vi "CilindarTest.vi"() -> ()   [LabVIEW 2014]
panel:
  out "Boolean 7":bool
  out "Boolean 6":bool
  out "Boolean 5":bool
  out "Boolean 4":bool
  out "Boolean 3":bool
  out "Boolean 2":bool
  out "Boolean":bool
  in  "stop":bool
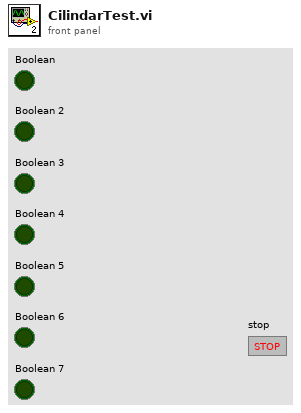
[diagram p1: front panel]
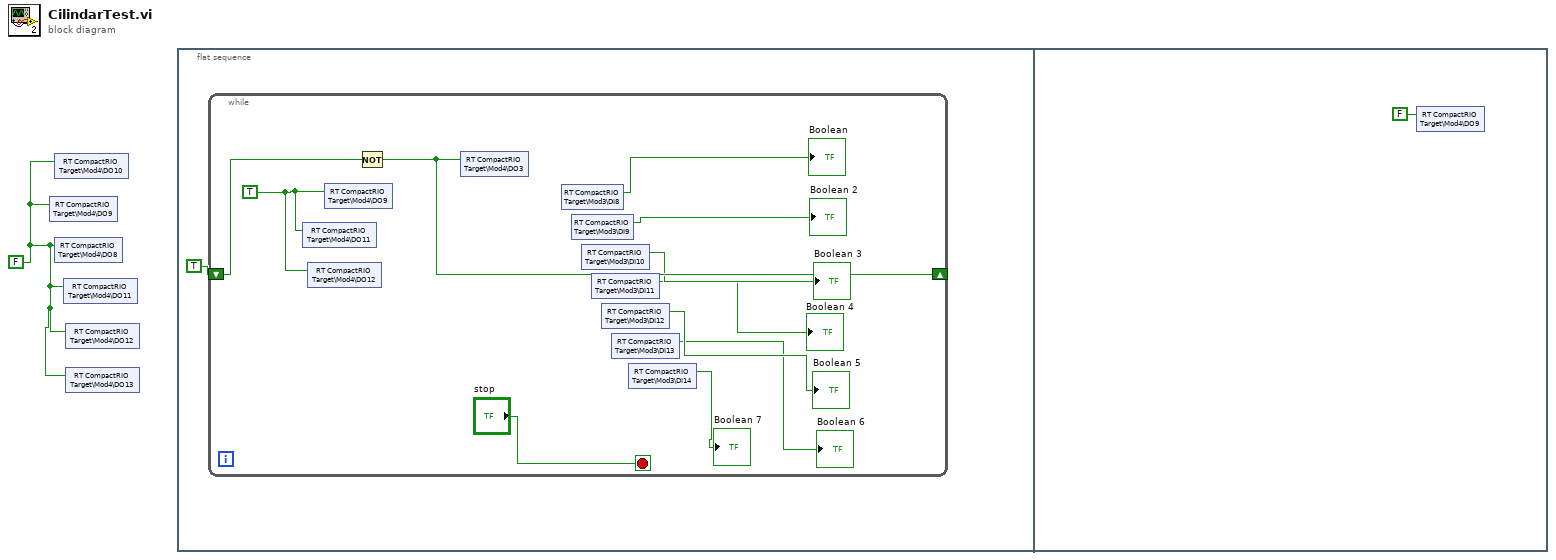
[diagram p0: block diagram]
diagram:
  w1 = FALSE
  n1 = shared-variable "RT CompactRIO Target\\Mod4\\DO9"(w1) -> ()  [unwired: 1 in, 1 out]
  n2 = shared-variable "RT CompactRIO Target\\Mod4\\DO10"(w1) -> ()  [unwired: 1 in, 1 out]
  n3 = shared-variable "RT CompactRIO Target\\Mod4\\DO8"(w1) -> ()  [unwired: 1 in, 1 out]
  n4 = shared-variable "RT CompactRIO Target\\Mod4\\DO11"(w1) -> ()  [unwired: 1 in, 1 out]
  n5 = shared-variable "RT CompactRIO Target\\Mod4\\DO12"(w1) -> ()  [unwired: 1 in, 1 out]
  n6 = shared-variable "RT CompactRIO Target\\Mod4\\DO13"(w1) -> ()  [unwired: 1 in, 1 out]
  n7 = flat-sequence {
    frame #0 {
      n8 = while {
        shift-right: [w12] -> _
        shift-left: TRUE ("DO8") -> [w13]
        stop <- "stop" stop-if-true
        w11 = TRUE ("DO8")
        n9 = shared-variable "RT CompactRIO Target\\Mod4\\DO11"(w11) -> ()  [unwired: 1 in, 1 out]
        n10 = shared-variable "RT CompactRIO Target\\Mod4\\DO12"(w11) -> ()  [unwired: 1 in, 1 out]
        n11 = shared-variable "RT CompactRIO Target\\Mod4\\DO9"(w11) -> ()  [unwired: 1 in, 1 out]
        n12 = Not(x=w13) -> (.not. x?=w12:bool)
        n13 = shared-variable "RT CompactRIO Target\\Mod4\\DO3"(w12) -> ()  [unwired: 1 in, 1 out]
        n14 = shared-variable "RT CompactRIO Target\\Mod3\\DI8"() -> (→"Boolean":bool)  [unwired: 1 in, 1 out]
        n15 = shared-variable "RT CompactRIO Target\\Mod3\\DI9"() -> (→"Boolean 2":bool)  [unwired: 1 in, 1 out]
        n16 = shared-variable "RT CompactRIO Target\\Mod3\\DI10"() -> (→"Boolean 3":bool)  [unwired: 1 in, 1 out]
        n17 = shared-variable "RT CompactRIO Target\\Mod3\\DI11"() -> (→"Boolean 4":bool)  [unwired: 1 in, 1 out]
        n18 = shared-variable "RT CompactRIO Target\\Mod3\\DI12"() -> (→"Boolean 5":bool)  [unwired: 1 in, 1 out]
        n19 = shared-variable "RT CompactRIO Target\\Mod3\\DI13"() -> (→"Boolean 6":bool)  [unwired: 1 in, 1 out]
        n20 = shared-variable "RT CompactRIO Target\\Mod3\\DI14"() -> (→"Boolean 7":bool)  [unwired: 1 in, 1 out]
      }
    }
    frame #1 {
      n21 = shared-variable "RT CompactRIO Target\\Mod4\\DO9"(FALSE ("DO8")) -> ()  [unwired: 1 in, 1 out]
    }
  }
